vi "Update Attributes A.vi"(7 "Attributes in":refnum<class "Attributes.lvclass">, 9 "VI Ref":refnum<vi>, 10 "Transport":refnum<class "Transport.lvclass">) -> (0 "Error out":errorcluster, 5 "Attributes out":refnum<class "Attributes.lvclass">)   [LabVIEW 2020, in "jettl.lvlib"]
uses:
  jettl.lvlib
  Attributes/Attributes.lvclass
  Transport/Transport.lvclass
  Attributes.ctl
  Msgs.ctl
  Msg/Msg.lvclass
  Actor/Actor.lvclass
  Base Attributes/Base Attributes/Base Attributes.lvclass/Base Attributes.ctl
  Base Attributes/Base Attributes/Base Attributes.lvclass
  C:/git/jettl/src/jettl/jettl/Attributes/Attributes.lvclass
  Base Attributes/Base Attributes.lvlib
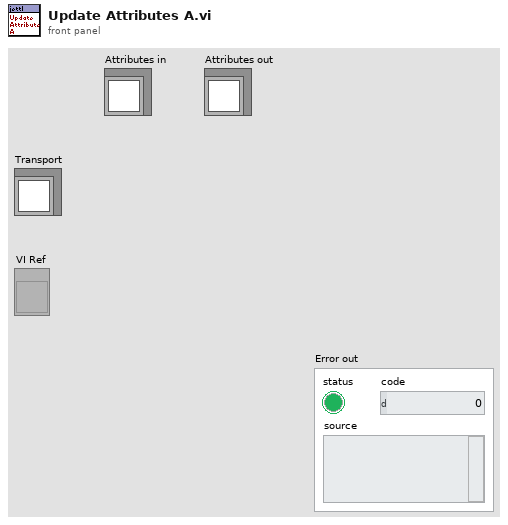
[diagram p1: front panel]
types:
  T1 = typedef "jettl.lvlib/Attributes.ctl" = cluster{"Unified Msgs":T2, "Edge Actors":refnum<class "Actor.lvclass">[], "Core Actors":refnum<class "Actor.lvclass">[], "Parent Attributes":refnum<class "Attributes.lvclass">, "Root":bool, "App Ref":refnum<vi>, "UID":string, "Transport":refnum<class "Transport.lvclass">, "VI Ref":refnum<vi>, "Actors":refnum<class "Actor.lvclass">[]}
  T2 = typedef "jettl.lvlib/Msgs.ctl" = set{refnum<class "Msg.lvclass">}
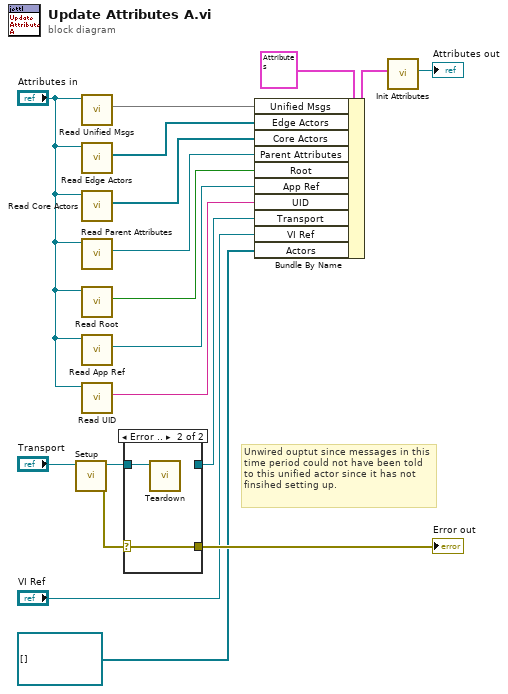
[diagram p0: block diagram]
diagram:
  # "Unwired ouptut since messages in this time period could not have been told to this unified actor since it has not finsihed setting up."
  n1 = call-dynamic "Setup.vi"("Transport in"="Transport") -> ("Error out"=w16:errorcluster, "Transport out"=w15:refnum<class "Transport.lvclass">)  [unwired: 9 in]
  n2 = call-dynamic "Read Unified Msgs.vi"("Attributes in"="Attributes in") -> ("Unified Msgs"=w3:T2)  [unwired: 10 in]
  n3 = call-dynamic "Read Edge Actors.vi"("Attributes in"="Attributes in") -> ("Edge Actors"=w2:refnum<class "Actor.lvclass">[])  [unwired: 10 in]
  n4 = call-dynamic "Read Core Actors.vi"("Attributes in"="Attributes in") -> ("Core Actors"=w8:refnum<class "Actor.lvclass">[])  [unwired: 10 in]
  n5 = call-dynamic "Read Parent Attributes.vi"("Attributes in"="Attributes in") -> ("Parent Attributes"=w9:refnum<class "Attributes.lvclass">)  [unwired: 10 in]
  n6 = call-dynamic "Read Root.vi"("Attributes in"="Attributes in") -> ("Root"=w10:bool)  [unwired: 10 in]
  n7 = call-dynamic "Read App Ref.vi"("Attributes in"="Attributes in") -> ("App Ref"=w11:refnum<vi>)  [unwired: 10 in]
  n8 = call-dynamic "Read UID.vi"("Attributes in"="Attributes in") -> ("UID"=w12:string)  [unwired: 10 in]
  n9 = case shown="Error .." w16 {
    selector: w16 -> [_ w20]
    tunnel: w15 -> [w19 w21]
    tunnel: [_ w20] -> w17
    tunnel: [w19 _] -> w4
    frame No Error {
    }
    frame Error {
      n10 = call-dynamic "Teardown.vi"("Transport in"=w21) -> ()  [unwired: 10 in, 1 out]
    }
  }
  "Error out" <- w17
  n11 = Bundle By Name(cluster=T1 {"Unified Msgs"={}, "Edge Actors"=[], "Core Actors"=[], "Parent Attributes"=refnum, "Root"=FALSE, "App Ref"=refnum, "UID"="", "Transport"=refnum, "VI Ref"=refnum, "Actors"=[]} ("Attributes"), "Unified Msgs"=w3, "Edge Actors"=w2, "Core Actors"=w8, "Parent Attributes"=w9, "Root"=w10, "App Ref"=w11, "UID"=w12, "Transport"=w4, "VI Ref"="VI Ref", "Actors"=refnum<class "Actor.lvclass">[] []) -> (w13:T1)
  n12 = call "Init Attributes.vi"("Attributes"=w13) -> ("Attributes"=→"Attributes out":refnum<class "Attributes.lvclass">)  [unwired: 10 in]
